vi "Clear.vi"(8 "error in (no error)":errorcluster, 11 "SQLite Connection In":refnum<class "Connection.lvclass">) -> (0 "error out":errorcluster, 3 "SQLite Connection Out":refnum<class "Connection.lvclass">)   [LabVIEW 2024, in "DBMigrations.lvlib"]
doc: "Delete all data in all tables in DB and reset autoincrement"
uses:
  DBMigrations.lvlib
  <vilib>/drjdpowell/SQLite Library/SQL Connection/Connection.lvclass
  <vilib>/drjdpowell/SQLite Library/SQL Connection/Execute SQL (No results).vi
  <vilib>/drjdpowell/SQLite Library/SQL Connection/Execute SQL (Single String).vi
  <vilib>/drjdpowell/SQLite Library/SQLite.lvlib
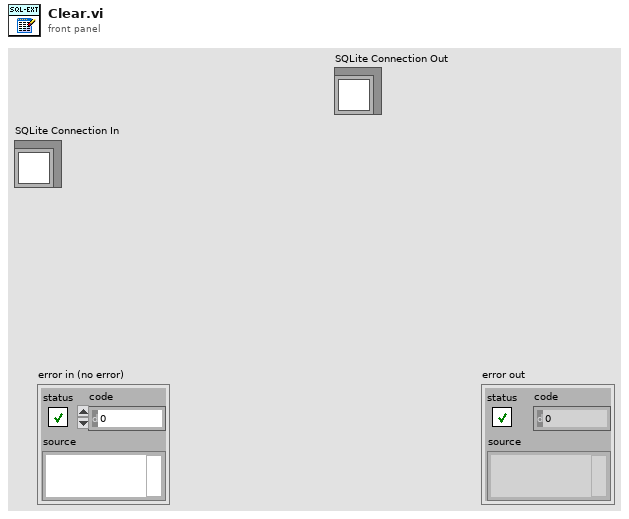
[diagram p1: front panel]
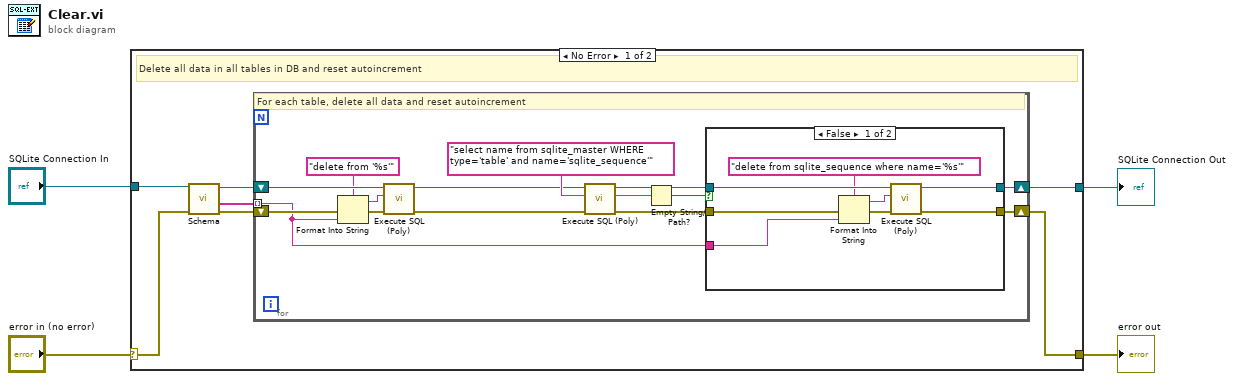
[diagram p0: block diagram]
diagram:
  n1 = case shown="No Error" "error in (no error)" {
    selector: "error in (no error)" -> [w10 w38]
    tunnel: [w11 w38] -> w3
    tunnel: "SQLite Connection In" -> [w7 w37]
    tunnel: [w5 w37] -> w1
    frame No Error {
      # "Delete all data in all tables in DB and reset autoincrement"
      n2 = call "Schema.vi"("error in (no error)"=w10, "SQLite Connection In"=w7) -> ("error out"=w9:errorcluster, "Table Names"=w8:string[], "SQLite Connection Out"=w6:refnum<class "Connection.lvclass">)  [unwired: 6 in, 1 out]
      n3 = for {
        shift-right: [w25] -> w11
        shift-left: w9 -> [w23]
        shift-right: [w26] -> w5
        shift-left: w6 -> [w24]
        tunnel: w8 -> [w19] mode=indexing
        # "For each table, delete all data and reset autoincrement"
        n4 = Format Into String(format string="delete from '%s'", error in=w23, w19) -> (resulting string=w20:string, error out=w22:errorcluster)  [unwired: 1 in]
        n5 = call-poly <vilib>:"Execute SQL (Poly).vi"("error in (no error)"=w22, "SQL"=w20, "SQLite Connection in"=w24) -> ("error out"=w15:errorcluster, "SQLite Connection"=w16:refnum<class "Connection.lvclass">)  [unwired: 7 in]
        n6 = call-poly <vilib>:"Execute SQL (Poly).vi"("error in (no error)"=w15, "SQL"="select name from sqlite_master WHERE type='table' and name='sqlite_sequence'", "SQLite Connection in"=w16) -> ("error out"=w14:errorcluster, "Result"=w18:string, "SQLite Connection"=w13:refnum<class "Connection.lvclass">)  [unwired: 6 in]
        n7 = Empty String/Path?(string/path=w18) -> (empty?=w12:bool)
        n8 = case shown="False" w12 {
          tunnel: [w34 w36] -> w26
          tunnel: [w33 w35] -> w25
          tunnel: w13 -> [w32 w36]
          tunnel: w14 -> [w31 w35]
          tunnel: w19 -> [w27 _]
          frame False {
            n9 = Format Into String(format string="delete from sqlite_sequence where name='%s'", error in=w31, w27) -> (resulting string=w28:string, error out=w30:errorcluster)  [unwired: 1 in]
            n10 = call-poly <vilib>:"Execute SQL (Poly).vi"("error in (no error)"=w30, "SQL"=w28, "SQLite Connection in"=w32) -> ("error out"=w33:errorcluster, "SQLite Connection"=w34:refnum<class "Connection.lvclass">)  [unwired: 7 in]
          }
          frame True {
          }
        }
      }
    }
    frame Error {
    }
  }
  "error out" <- w3
  "SQLite Connection Out" <- w1
